vi "table_set_subtable_item.vi"(4 "subkeys":string[](array[string]), 6 "close_item? (true)":bool=TRUE, 7 "subtables":string[](array[string]), 8 "error in (no error)":errorcluster, 9 "item (value)":refnum<class "Item.lvclass">, 10 "key":string, 11 "Table in":refnum<class "Table.lvclass">) -> (0 "error out":errorcluster, 3 "Table out":refnum<class "Table.lvclass">)   [LabVIEW 2020, in "toml.lvclass"]
uses:
  toml.lvclass
  Item/Item.lvclass
  Table/Table.lvclass
  InlineTable/InlineTable.lvclass
  Value/Value.lvclass
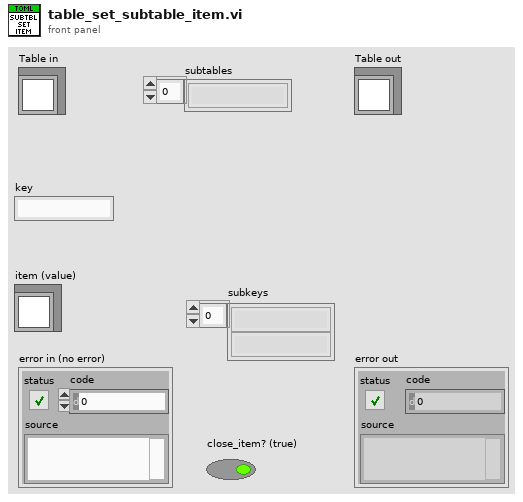
[diagram p1: front panel]
types:
  T1 = typedef "toml_edit.lvlib/Item.lvclass/type--enum.ctl" = enum16{"Unknown", "None", "Value", "ArrayOfTables", "Table"}
  T2 = typedef "toml_edit.lvlib/Value.lvclass/value_type--enum.ctl" = enum16{"Unknown", "String", "Integer", "Float", "Boolean", "Datetime", "Array", "InlineTable"}
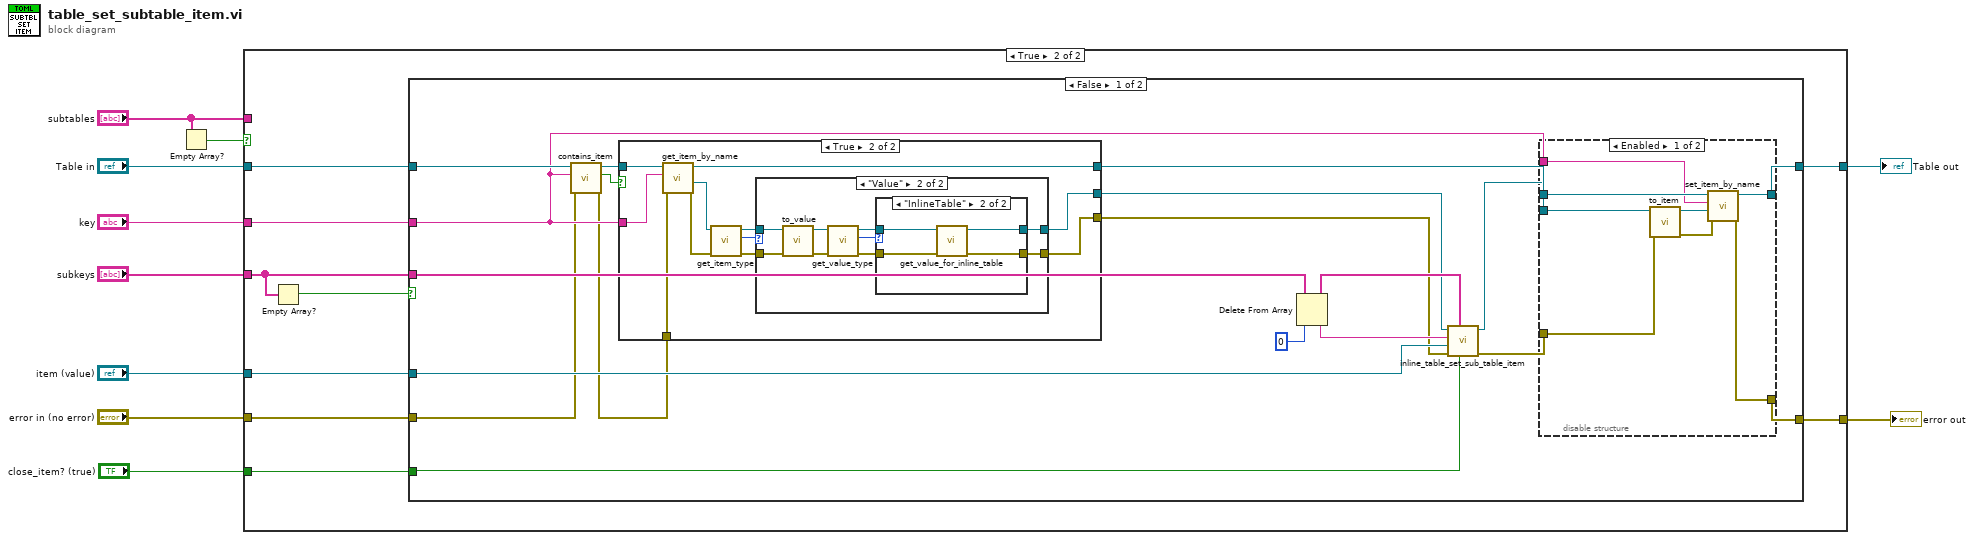
[diagram p0: block diagram]
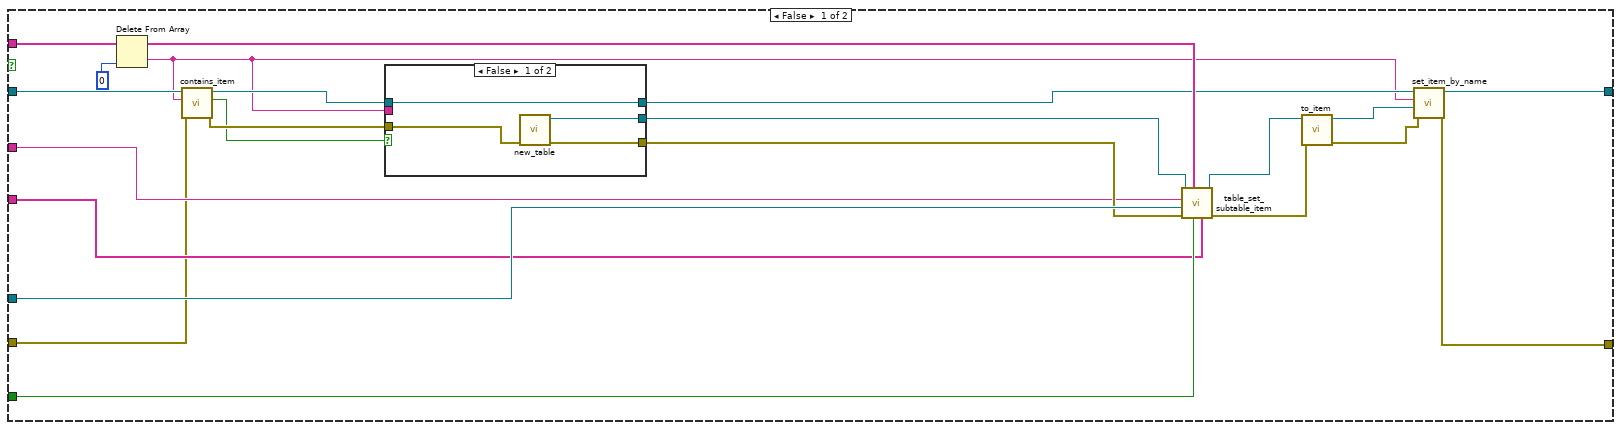
[diagram p2: hidden frame]
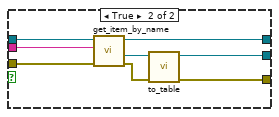
[diagram p3: hidden frame]
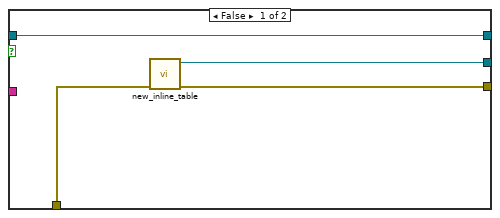
[diagram p4: hidden frame]
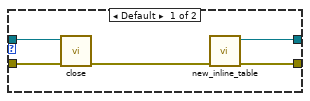
[diagram p5: hidden frame]
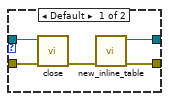
[diagram p6: hidden frame]
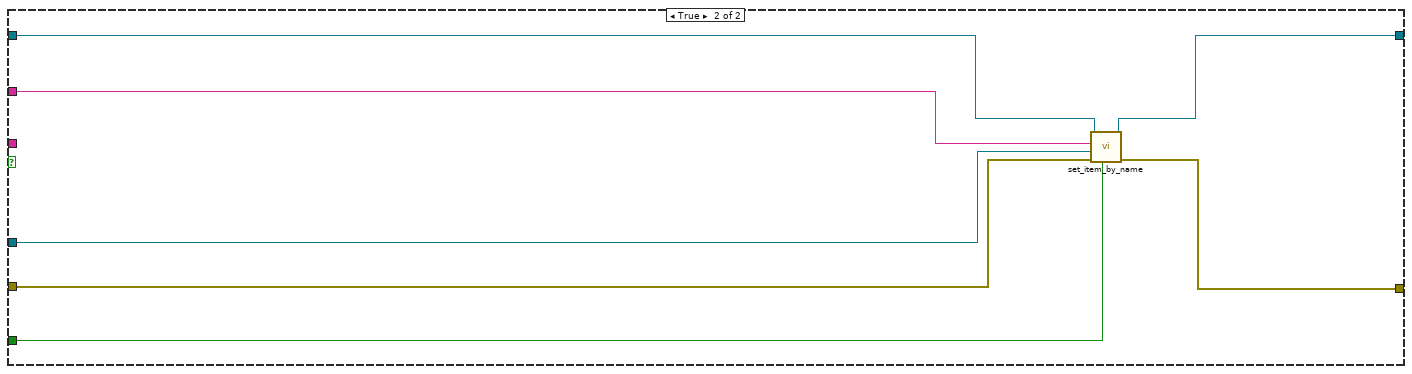
[diagram p8: hidden frame]
diagram:
  n1 = Empty Array?(array="subtables") -> (empty?=w4:bool)
  n2 = case shown="True" w4 {
    tunnel: [w25 w53] -> w10
    tunnel: "item (value)" -> [w27 w50]
    tunnel: "subkeys" -> [w18 w46]
    tunnel: [w21 w52] -> w7
    tunnel: "Table in" -> [w16 w51]
    tunnel: "error in (no error)" -> [w14 w49]
    tunnel: "subtables" -> [w32 _]
    tunnel: "close_item? (true)" -> [w20 w48]
    tunnel: "key" -> [w19 w45]
    frame False {
      n3 = Delete From Array(array=w32, index=0) -> (deleted portion=w13:string, array with subset deleted=w30:string[])  [unwired: 1 in]
      n4 = call "contains_item.vi"("error in (no error)"=w14, "item_name"=w13, "Table in"=w16) -> ("error out"=w15:errorcluster, "contains_item"=w12:bool, "Table out"=w17:refnum<class "Table.lvclass">)  [unwired: 6 in]
      n5 = case shown="False" w12 {
        tunnel: [w35 w44] -> w29
        tunnel: [w36 w43] -> w28
        tunnel: [w33 w42] -> w26
        tunnel: w17 -> [w35 w41]
        tunnel: w15 -> [w34 w40]
        tunnel: w13 -> [_ w39]
        frame False {
          n6 = call "new_table.vi"("error in (no error)"=w34) -> ("error out"=w33:errorcluster, "Table out"=w36:refnum<class "Table.lvclass">)  [unwired: 9 in]
        }
        frame True {
          n7 = call "get_item_by_name.vi"("error in (no error)"=w40, "item_name"=w39, "Table in"=w41) -> ("error out"=w37:errorcluster, "Item"=w38:refnum<class "Item.lvclass">, "Table out"=w44:refnum<class "Table.lvclass">)  [unwired: 4 in, 2 out]
          n8 = call "to_table.vi"("error in (no error)"=w37, "Item in"=w38) -> ("error out"=w42:errorcluster, "Table"=w43:refnum<class "Table.lvclass">)  [unwired: 8 in]
        }
      }
      n9 = call "table_set_subtable_item.vi"("subkeys"=w18, "close_item? (true)"=w20, "subtables"=w30, "error in (no error)"=w26, "item (value)"=w27, "key"=w19, "Table in"=w28) -> ("error out"=w23:errorcluster, "Table out"=w24:refnum<class "Table.lvclass">)  [unwired: 3 in]
      n10 = call "to_item.vi"("error in (no error)"=w23, "Table in"=w24) -> ("error out"=w22:errorcluster, "Item out"=w11:refnum<class "Item.lvclass">)  [unwired: 8 in]
      n11 = call "set_item_by_name.vi"("error in (no error)"=w22, "Item"=w11, "item_name"=w13, "Table in"=w29) -> ("error out"=w25:errorcluster, "Table out"=w21:refnum<class "Table.lvclass">)  [unwired: 6 in]
    }
    frame True {
      n12 = Empty Array?(array=w46) -> (empty?=w47:bool)
      n13 = case shown="False" w47 {
        tunnel: [w63 w127] -> w53
        tunnel: [w64 w126] -> w52
        tunnel: w51 -> [w58 w125]
        tunnel: w50 -> [w65 w124]
        tunnel: w49 -> [w55 w123]
        tunnel: w48 -> [w62 w122]
        tunnel: w46 -> [w67 _]
        tunnel: w45 -> [w57 w121]
        frame False {
          n14 = call "contains_item.vi"("error in (no error)"=w55, "item_name"=w57, "Table in"=w58) -> ("error out"=w56:errorcluster, "contains_item"=w54:bool, "Table out"=w59:refnum<class "Table.lvclass">)  [unwired: 6 in]
          n15 = case shown="True" w54 {
            tunnel: [w73 w85] -> w72
            tunnel: [w74 w77] -> w61
            tunnel: [w76 w79] -> w60
            tunnel: w59 -> [w73 w87]
            tunnel: w57 -> [_ w84]
            tunnel: w56 -> [w75 w86]
            frame False {
              n16 = call "new_inline_table.vi"("error in (no error)"=w75) -> ("error out"=w74:errorcluster, "InlineTable out"=w76:refnum<class "InlineTable.lvclass">)  [unwired: 9 in]
            }
            frame True {
              n17 = call "get_item_by_name.vi"("error in (no error)"=w86, "item_name"=w84, "Table in"=w87) -> ("error out"=w78:errorcluster, "Item"=w83:refnum<class "Item.lvclass">, "Table out"=w85:refnum<class "Table.lvclass">)  [unwired: 4 in, 2 out]
              n18 = call "get_item_type.vi"("error in (no error)"=w78, "Item in"=w83) -> ("error out"=w80:errorcluster, "item_type"=w82:T1, "Item out"=w81:refnum<class "Item.lvclass">)  [unwired: 7 in]
              n19 = case shown="\"Value\"" w82 {
                tunnel: w81 -> [w89 w101]
                tunnel: w80 -> [w90 w98]
                tunnel: [w91 w94] -> w79
                tunnel: [w92 w93] -> w77
                frame Default {
                  n20 = call "close.vi"("error in (no error)"=w90, "Item in"=w89) -> ("error out"=w88:errorcluster)  [unwired: 9 in]
                  n21 = call "new_inline_table.vi"("error in (no error)"=w88) -> ("error out"=w92:errorcluster, "InlineTable out"=w91:refnum<class "InlineTable.lvclass">)  [unwired: 9 in]
                }
                frame "Value" {
                  n22 = call "to_value.vi"("error in (no error)"=w98, "Item in"=w101) -> ("error out"=w100:errorcluster, "Value out"=w99:refnum<class "Value.lvclass">)  [unwired: 8 in]
                  n23 = call "get_value_type.vi"("error in (no error)"=w100, "Value in"=w99) -> ("error out"=w95:errorcluster, "value_type"=w97:T2, "Value out"=w96:refnum<class "Value.lvclass">)  [unwired: 7 in]
                  n24 = case shown="\"InlineTable\"" w97 {
                    tunnel: w96 -> [w104 w110]
                    tunnel: w95 -> [w103 w109]
                    tunnel: [w106 w108] -> w94
                    tunnel: [w105 w107] -> w93
                    frame Default {
                      n25 = call "close.vi"("error in (no error)"=w103, "Value in"=w104) -> ("error out"=w102:errorcluster)  [unwired: 9 in]
                      n26 = call "new_inline_table.vi"("error in (no error)"=w102) -> ("error out"=w105:errorcluster, "InlineTable out"=w106:refnum<class "InlineTable.lvclass">)  [unwired: 9 in]
                    }
                    frame "InlineTable" {
                      n27 = call "get_value_for_inline_table.vi"("error in (no error)"=w109, "Value in"=w110) -> ("error out"=w107:errorcluster, "InlineTable out"=w108:refnum<class "InlineTable.lvclass">)  [unwired: 8 in]
                    }
                  }
                }
              }
            }
          }
          n28 = Delete From Array(array=w67, index=0) -> (deleted portion=w66:string, array with subset deleted=w68:string[])  [unwired: 1 in]
          n29 = call "inline_table_set_sub_table_item.vi"("close_item? (true)"=w62, "subtables"=w68, "error in (no error)"=w61, "item (value)"=w65, "key"=w66, "InlineTable in"=w60) -> ("error out"=w71:errorcluster, "InlineTable out"=w70:refnum<class "InlineTable.lvclass">)  [unwired: 4 in]
          n30 = disable-structure shown="Enabled" {
            disable-tunnel: w72 -> [w118 w120]
            disable-tunnel: [w117 w120] -> w64
            disable-tunnel: [w116 w119] -> w63
            disable-tunnel: w71 -> [w115 w119]
            disable-tunnel: w70 -> [w114 _]
            disable-tunnel: w57 -> [w113 _]
            frame Enabled {
              n31 = call "to_item.vi"("error in (no error)"=w115, "Table in"=w114) -> ("error out"=w112:errorcluster, "Item out"=w111:refnum<class "Item.lvclass">)  [unwired: 8 in]
              n32 = call "set_item_by_name.vi"("error in (no error)"=w112, "Item"=w111, "item_name"=w113, "Table in"=w118) -> ("error out"=w116:errorcluster, "Table out"=w117:refnum<class "Table.lvclass">)  [unwired: 6 in]
            }
            frame Disabled {
            }
          }
        }
        frame True {
          n33 = call "set_item_by_name.vi"("close_item? (true)"=w122, "error in (no error)"=w123, "Item"=w124, "item_name"=w121, "Table in"=w125) -> ("error out"=w127:errorcluster, "Table out"=w126:refnum<class "Table.lvclass">)  [unwired: 5 in]
        }
      }
    }
  }
  "error out" <- w10
  "Table out" <- w7
